vi "macro_MatBuilder_Create.vi"   [LabVIEW 2019, in "Trajectory_Library.lvlib"]
uses:
  Trajectory_Library.lvlib
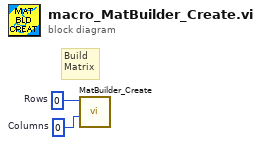
[diagram p0: block diagram]
diagram:
  w1 = 0  # Columns
  w2 = 0  # Rows
  # "Build\nMatrix"
  n1 = call "MatBuilder_Create.vi"("Columns"=w1, "Rows"=w2) -> ()  [unwired: 9 in, 1 out]
